vi "Build Progress Event.vi"(8 "message":string, 9 "total":dbl=nan, 10 "progress":dbl, 11 "progressToken":string) -> (3 "event":string)   [LabVIEW 2020, in "MCP Server.lvlib"]
doc: "Builds the Server-Sent Event that Report Progress.vi sends: data: {\"jsonrpc\":\"2.0\",\"method\":\"notifications/progress\",\"params\":{\"progressToken\":..,\"progress\":..,\"total\":..,\"message\":..}} followed by a blank line.\n\ntotal is left out when it is NaN or not greater than 0, message when it is empty."
uses:
  MCP Server.lvlib
  613cbc13-1098-4f58-bebf-b43248a25ef1.vi
  1372a7ff-d8c0-49b1-9d08-3c4996c0f9ff.vi
  fb32823f-c1c4-49b6-b7c4-df1dbf3f17fb.vi
  <vilib>/JDP Science/JSONtext/Variant to JSON Text.vi
  <vilib>/JDP Science/JSONtext/LVClass Serializer/JSONtext LVClass Serializer.lvclass
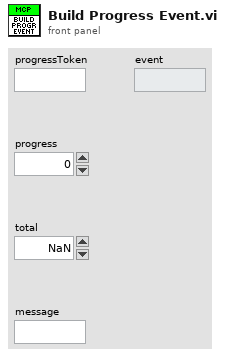
[diagram p1: front panel]
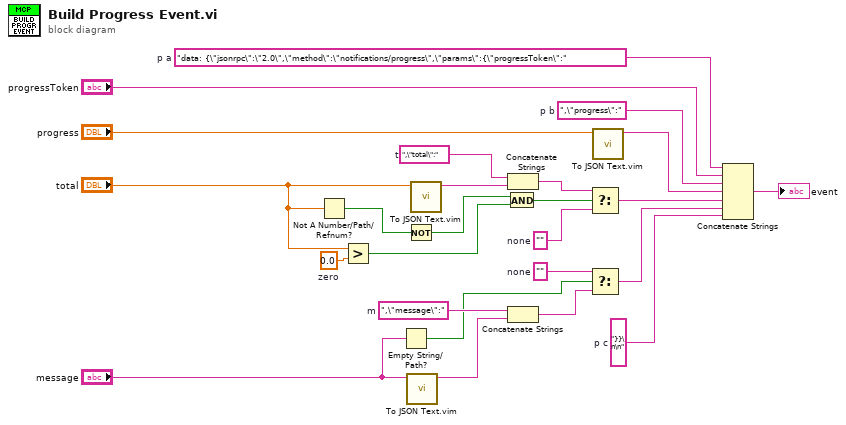
[diagram p0: block diagram]
diagram:
  w11 = ""  # none
  w15 = ""  # none
  w22 = 0.0  # zero
  w13 = ",\"message\":"  # m
  w19 = ",\"total\":"  # t
  w2 = "}}\n\n"  # p c
  w6 = ",\"progress\":"  # p b
  w8 = "data: {\"jsonrpc\":\"2.0\",\"method\":\"notifications/progress\",\"params\":{\"progressToken\":"  # p a
  n1 = Not A Number/Path/Refnum?(number/path/refnum="total") -> (NaN/Path/Refnum?=w24:bool)
  n2 = Greater?(x="total", y=w22) -> (0:w20:bool)
  n3 = Empty String/Path?(string/path="message") -> (empty?=w10:bool)
  n4 = Not(x=w24) -> (.not. x?=w21:bool)
  n5 = call "To JSON Text.vim"("Anything"="message") -> ("<JSON>"=w12:string)  [unwired: 9 in, 1 out]
  n6 = call "To JSON Text.vim"("Anything"="total") -> ("<JSON>"=w18:string)  [unwired: 9 in, 1 out]
  n7 = And(x=w21, y=w20) -> (x .and. y?=w16:bool)
  n8 = Concatenate Strings(w19, w18) -> (w17:string)
  n9 = Concatenate Strings(w13, w12) -> (w9:string)
  n10 = Select(t=w17, s=w16, f=w15) -> (s? t:f=w4:string)
  n11 = Select(t=w11, s=w10, f=w9) -> (s? t:f=w3:string)
  n12 = call "To JSON Text.vim"("Anything"="progress") -> ("<JSON>"=w5:string)  [unwired: 9 in, 1 out]
  n13 = Concatenate Strings(w8, "progressToken", w6, w5, w4, w3, w2) -> (→"event":string)
